vi "LoadTbl9 (SubVI).vi"(8 "error in":errorcluster, 11 "Log":refnum<vi>) -> (0 "error out":errorcluster, 3 "Array":sgl[][](array[numeric]))   [LabVIEW 2017]
uses:
  Global_SNK3_HF.vi
  LV_Unicorn/LV_Unicorn.lvlib
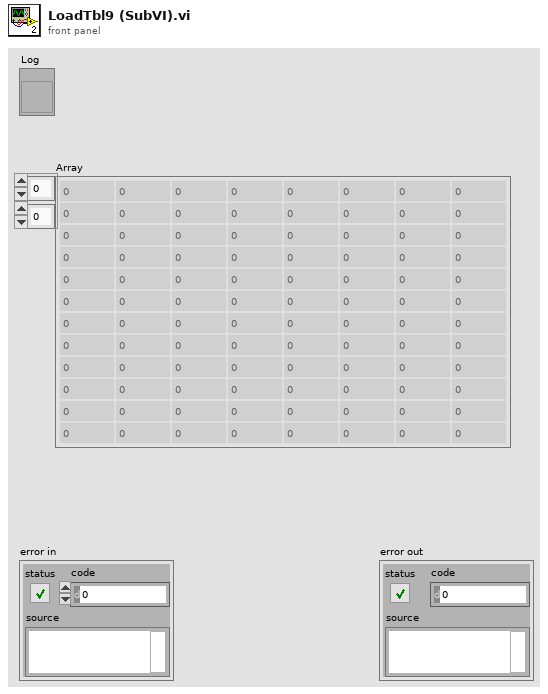
[diagram p1: front panel]
types:
  T1 = typedef "LV_Unicorn.lvlib/unicorn_Param.ctl" = cluster{"conParam":T2, "Param":T3}
  T2 = typedef "LV_Unicorn.lvlib/unicorn_conn.ctl" = cluster{"ReadIntParam":bool, "ReadDescrParam":bool, "ReadFloatParam":bool, "debug":bool, "ReadJSON":bool, "IP_address":string, "N_attempts":i32, "type_con":enum16{"Serial", "TCP"}, "MB_address":i32, "VISA":refnum<visa-resource-name>, "connection ID":refnum<k5>, "nameDevices":string, "timeout":i32, "port":u16, "type_version":string, "baud_rate":u32, "VersionControl":bool, "TCP_conn":bool, "WindowSize":i32}
  T3 = typedef "LV_Unicorn.lvlib/unicorn_JSON.ctl" = cluster{"NumParam":cluster{"NTelem":i32, "NInt":i32, "NFloat":i32, "NTable":i32}, "ParamInt":T4, "Telemetry":T5, "Table":T6, "ParamFloat":T7}
  T4 = typedef "LV_Unicorn.lvlib/unicorn_ParamInt.ctl" = cluster{"ID":string, "Num":i32, "Name":string, "Type":string, "Enum":string, "Desc":string, "Unit":string, "Access":string, "FormatStr":string, "Min":i32, "Max":i32}[]
  T5 = typedef "LV_Unicorn.lvlib/unicorn_Telemetry.ctl" = cluster{"ID":string, "Num":i32, "Name":string, "Desc":string, "Unit":string, "FormatStr":string, "Min":i32, "Max":i32}[]
  T6 = typedef "LV_Unicorn.lvlib/unicorn_Table.ctl" = cluster{"Num":i32, "Access":string, "ColumnCount":i32, "NeedParamPrepare":bool, "Columns":cluster{"Column":i32, "Desc":string, "Name":string}[], "DataType":string, "FormatStr":string, "ID":string, "Name":string, "RowCount":i32, "Rows":cluster{"Desc":string, "ID":string, "Max":i32, "Min":i32, "Name":string, "Row":i32, "Unit":string}[], "Type":string}[]
  T7 = typedef "LV_Unicorn.lvlib/unicorn_ParamFloat.ctl" = cluster{"ID":string, "Num":i32, "Name":string, "Type":string, "Enum":string, "Desc":string, "Unit":string, "Access":string, "FormatStr":string, "Min":sgl, "Max":sgl}[]
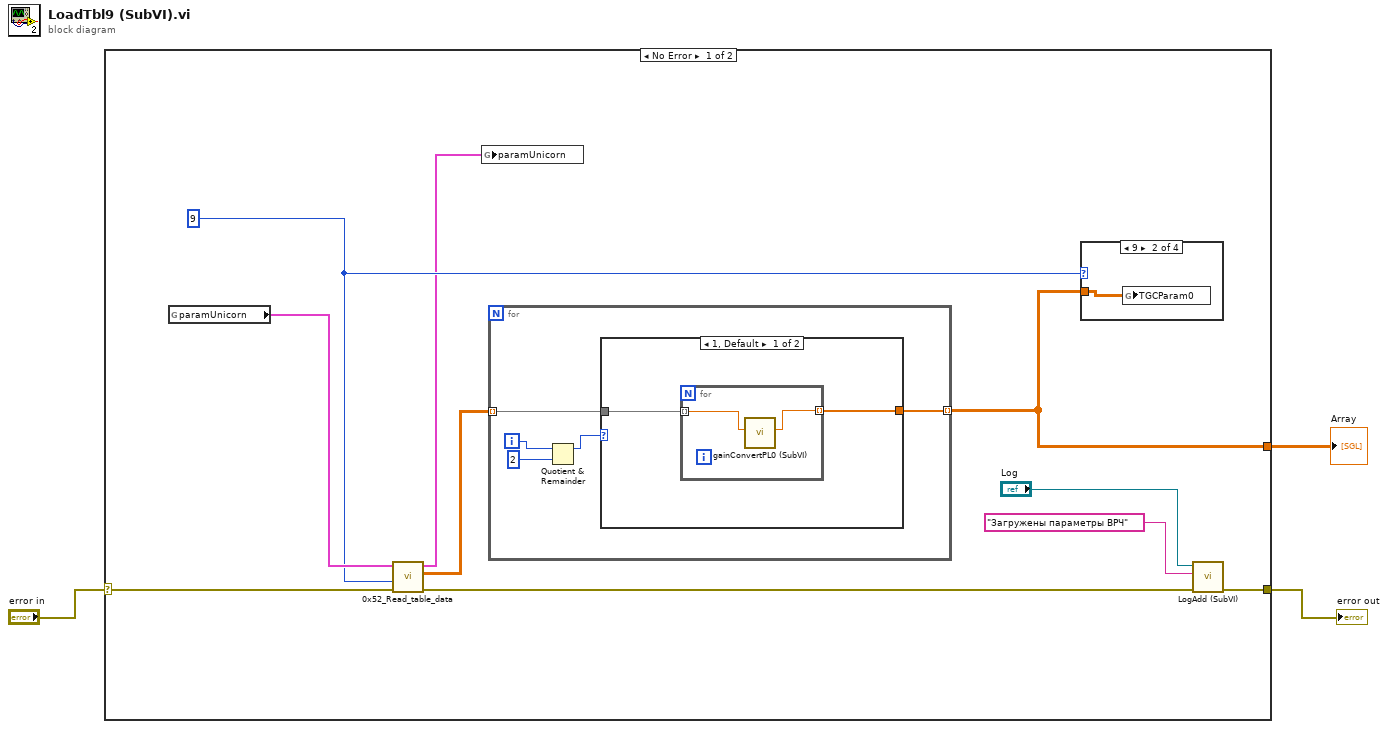
[diagram p0: block diagram]
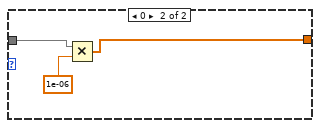
[diagram p2: hidden frame]
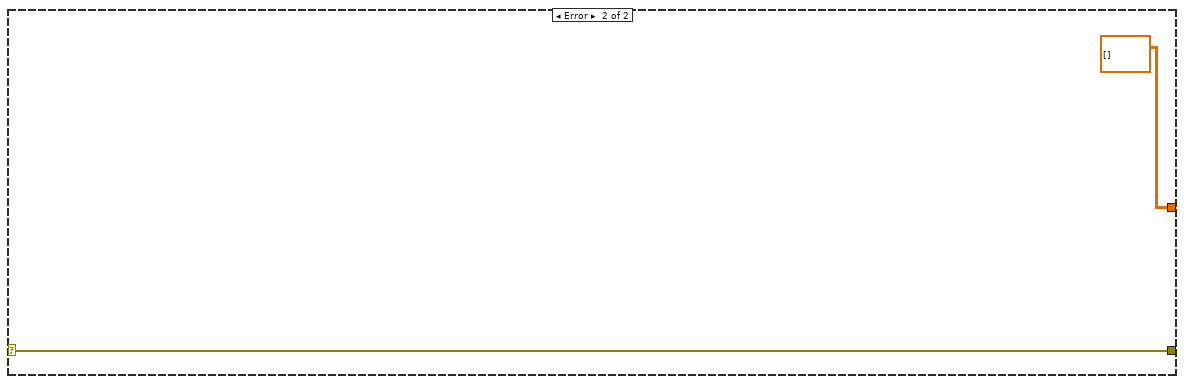
[diagram p6: hidden frame]
diagram:
  n1 = case shown="No Error" "error in" {
    selector: "error in" -> [w7 w27]
    tunnel: [w4 w27] -> w3
    tunnel: [w5 sgl[][] [] ("Array")] -> w2
    frame No Error {
      w10 = 9 ("NTable")
      n2 = global read "Global_SNK3_HF.vi" "paramUnicorn"() -> (w11:T1)
      n3 = call "0x52_Read_table_data.vi"("error in"=w7, "NTable"=w10, "paramUnicornIn"=w11) -> ("error out"=w9:errorcluster, "Array"=w6:sgl[][], "paramUnicornOut"=w8:T1)  [unwired: 6 in]
      n4 = global write "Global_SNK3_HF.vi" "paramUnicorn"(w8) -> ()
      n5 = for {
        tunnel: w6 -> [w15] mode=indexing
        tunnel: [w14] -> w5 mode=indexing
        i -> [w18]
        n6 = Quotient & Remainder(x=w18, y=2) -> (x-y*floor(x/y)=w16:i32)  [unwired: 1 out]
        n7 = case shown="1, Default" w16 {
          tunnel: w15 -> [w20 w25]
          tunnel: [w19 w24] -> w14
          frame 1, Default {
            n8 = for {
              tunnel: w20 -> [w22] mode=indexing
              tunnel: [w21] -> w19 mode=indexing
              n9 = call "gainConvertPL0 (SubVI).vi"("DACin"=w22) -> ("GainOUT"=w21:sgl)  [unwired: 8 in, 2 out]
            }
          }
          frame 0 {
            n10 = Multiply(x=w25, y=1e-06) -> (x*y=w24:dbl[])
          }
        }
      }
      n11 = case shown="9" w10 {
        tunnel: w5 -> [_ w26 _ _]
        frame 1 {
        }
        frame 9 {
          n12 = global write "Global_SNK3_HF.vi" "TGCParam0"(w26) -> ()
        }
        frame 2, Default {
        }
        frame 0 {
        }
      }
      n13 = call "LogAdd (SubVI).vi"("error in"=w9, "string"="Загружены параметры ВРЧ", "Log"="Log") -> ("error out"=w4:errorcluster)  [unwired: 8 in]
    }
    frame Error {
    }
  }
  "error out" <- w3
  "Array" <- w2
